vi "Gen_stop.vi"(8 "error in (no error)":errorcluster, 10 "Canal":u8, 11 "VISA resource name":refnum<visa-resource-name>) -> (0 "error out":errorcluster, 2 "ok":bool, 3 "VISA resource name out":refnum<visa-resource-name>)   [LabVIEW 2026]
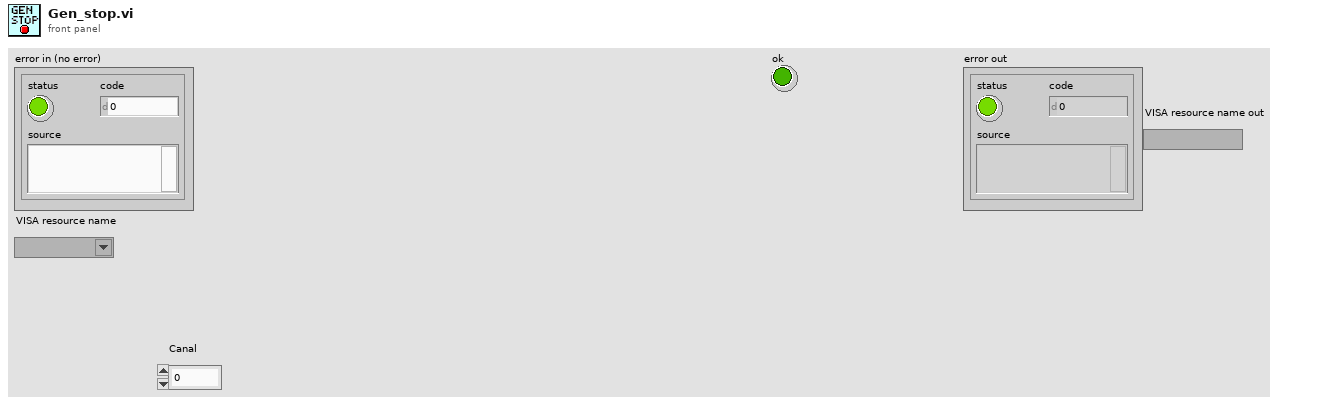
[diagram p1: front panel]
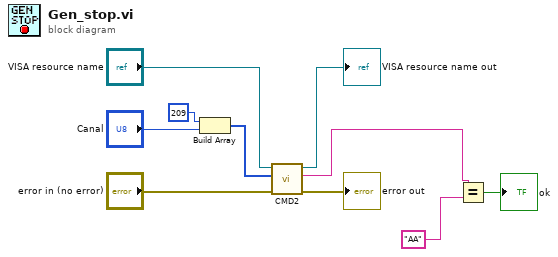
[diagram p0: block diagram]
diagram:
  n1 = Build Array(u8 209, "Canal") -> (w4:u8[])
  n2 = call "CMD2.vi"("error in (no error)"="error in (no error)", "Comando"=w4, "VISA resource name"="VISA resource name") -> ("error out"=→"error out":errorcluster, "respuesta"=w3:string, "VISA resource name out"=→"VISA resource name out":refnum<visa-resource-name>)  [unwired: 6 in]
  n3 = Equal?(x=w3, y="AA") -> (x = y?=→"ok":bool)
